vi "Create Folder Shot.vi"(6 "Folders to Exclude":string[](array[string]), 8 "error in (no error)":errorcluster, 10 "Log File Path (*.txt)":path, 11 "Directory Path":path) -> (0 "error out":errorcluster, 3 "Folder Shot":T1[](array[typedef]))   [LabVIEW 2016, in "SLL File IO.lvlib"]
doc: "Create a Folder Shot File for the provided Folder Path.\n\nFor each file, it calculates the CRC and stores them in the log file."
uses:
  SLL File IO.lvlib
  _Typedefs/Folder Shot Element.ctl
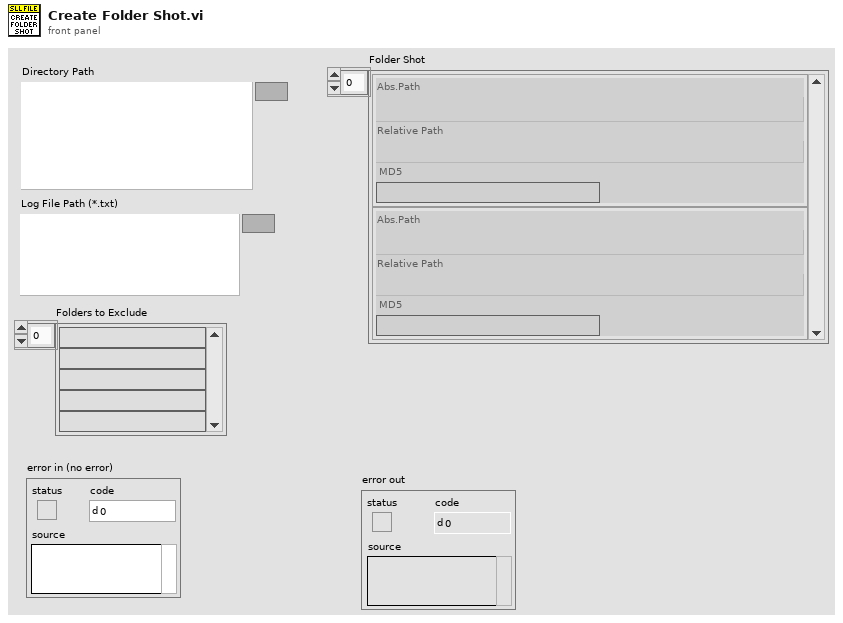
[diagram p1: front panel]
types:
  T1 = typedef "SLL File IO.lvlib/Folder Shot Element.ctl" = cluster{"Abs.Path":path, "Relative Path":path, "MD5":string}
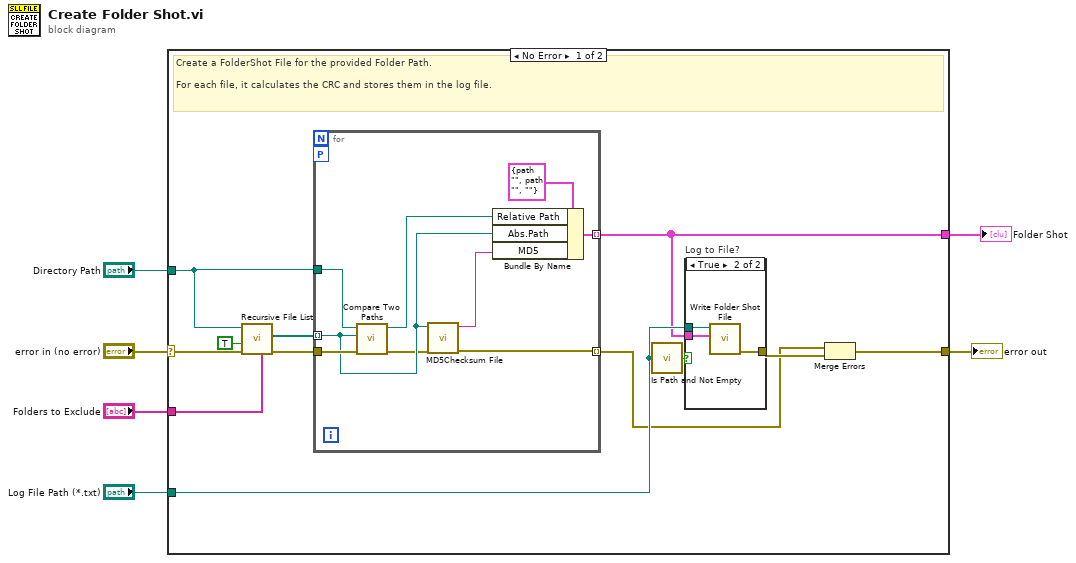
[diagram p0: block diagram]
diagram:
  n1 = case shown="No Error" "error in (no error)" {
    selector: "error in (no error)" -> [w18 w31]
    tunnel: [w8 w31] -> w5
    tunnel: "Directory Path" -> [w14 _]
    tunnel: [w10 _] -> w3
    tunnel: "Folders to Exclude" -> [w13 _]
    tunnel: "Log File Path (*.txt)" -> [w11 _]
    frame No Error {
      # "Create a FolderShot File for the provided Folder Path.\n\nFor each file, it calculates the CRC and stores them in the log file."
      n2 = call <vilib>:"Recursive File List.vi"("Folders to Exclude"=w13, "error in (no error)"=w18, "Continue Recursing on Error? (F)"=TRUE, "Folder Path"=w14) -> ("error out"=w16:errorcluster, "All Files in Dir"=w15:path[])  [unwired: 3 in, 3 out]
      n3 = for {
        tunnel: w15 -> [w26] mode=indexing
        tunnel: w14 -> [w30]
        tunnel: [w22] -> w10 mode=indexing
        workers-P: _ -> [_]
        tunnel: w16 -> [w27]
        tunnel: [w23] -> w7 mode=indexing
        n4 = call <vilib>:"Compare Two Paths.vi"("error in (no error)"=w27, "Path 2"=w26, "Path 1"=w30) -> ("error out"=w24:errorcluster, "Relative Path from 1 to 2"=w28:path)  [unwired: 5 in, 2 out]
        n5 = call <vilib>:"MD5Checksum File.vi"("error in (no error)"=w24, "Path"=w26) -> ("error out"=w23:errorcluster, "MD5 message-digest"=w25:string)  [unwired: 8 in]
        n6 = Bundle By Name(cluster=T1 {"Abs.Path"=path "", "Relative Path"=path "", "MD5"=""} ("Folder Shot Element"), "Relative Path"=w28, "Abs.Path"=w26, "MD5"=w25) -> (w22:T1)
      }
      n7 = call <vilib>:"Is Path and Not Empty.vi"("path"=w11) -> ("Is Path and Not Empty?"=w9:bool)  [unwired: 4 in]
      n8 = case "Log to File?" shown="True" w9 {
        tunnel: [_ w21] -> w12
        tunnel: w11 -> [_ w20]
        tunnel: w10 -> [_ w19]
        frame False {
        }
        frame True {
          n9 = call "Write Folder Shot File.vi"("Folder Shot"=w19, "Log Path"=w20) -> ("error out"=w21:errorcluster)  [unwired: 9 in]
        }
      }
      n10 = Merge Errors(w7, w12) -> (w8:errorcluster)
    }
    frame Error {
    }
  }
  "error out" <- w5
  "Folder Shot" <- w3
